vi "Colour to RGB.vi"(8 "error in (no error)":errorcluster, 11 "Colour":u32(colorbox)) -> (0 "error out":errorcluster, 1 "Blue":u8, 2 "Green":u8, 3 "Red":u8, 5 "Resolved Colour":u32 format="%.0x")   [LabVIEW 2018, in "Colour Lab.lvlib"]
uses:
  Colour Lab.lvlib
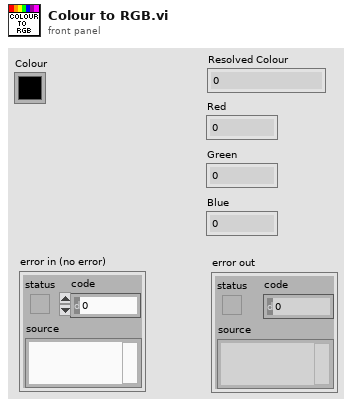
[diagram p1: front panel]
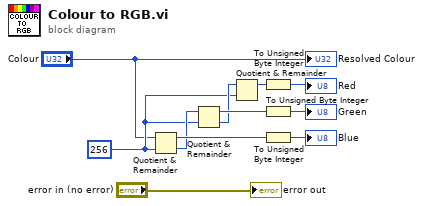
[diagram p0: block diagram]
diagram:
  w5 = u32 256 ("x")
  n1 = Quotient & Remainder(x="Colour", y=w5) -> (x-y*floor(x/y)=w10:u32, floor(x/y)=w9:u32)
  n2 = Quotient & Remainder(x=w9, y=w5) -> (x-y*floor(x/y)=w8:u32, floor(x/y)=w7:u32)
  n3 = Quotient & Remainder(x=w7, y=w5) -> (x-y*floor(x/y)=w6:u32)  [unwired: 1 out]
  n4 = To Unsigned Byte Integer(number=w6) -> (unsigned 8bit integer=→"Red":u8)
  n5 = To Unsigned Byte Integer(number=w8) -> (unsigned 8bit integer=→"Green":u8)
  n6 = To Unsigned Byte Integer(number=w10) -> (unsigned 8bit integer=→"Blue":u8)
  "Resolved Colour" <- "Colour"
  "error out" <- "error in (no error)"
